vi "process_exit_callback.vi"(4 "ProcessExit Event":refnum<user-event>, 5 "Event Data":cluster{"sender":refnum<k24>, "e":refnum<k24>}, 6 "Control Ref":refnum<k24>, 7 "Event Common Data":T1) -> ()   [LabVIEW 2021, in "dotnet_system_exec.lvclass"]
doc: "Process Exit Callback VI"
uses:
  dotnet_system_exec.lvclass
  ProcessExit Event.ctl
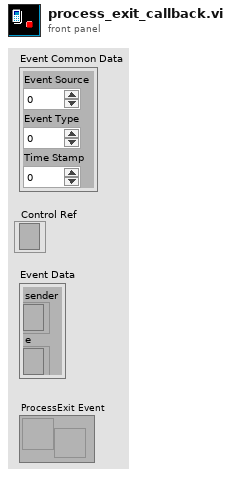
[diagram p1: front panel]
types:
  T1 = cluster{"Event Source":i32, "Event Type":u32, "Time Stamp":u32}
  T2 = typedef "dotnet_system_exec.lvclass/ProcessExit Event.ctl" = cluster{"HasExited":bool, "ExitCode":i32}
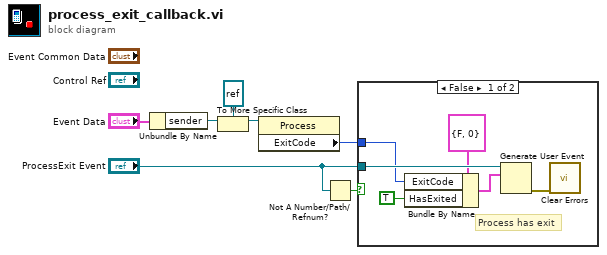
[diagram p0: block diagram]
diagram:
  n1 = Unbundle By Name("Event Data") -> ("sender"=w1:refnum<k24>)
  n2 = To More Specific Class(target class=refnum<k24> refnum ("Process Ref"), reference=w1) -> (specific class reference=w4:refnum<k24>)  [unwired: 1 in, 1 out]
  n3 = property class="Process"(reference=w4) -> ("ExitCode"=w2:i32)  [unwired: 1 in, 2 out]
  n4 = Not A Number/Path/Refnum?(number/path/refnum="ProcessExit Event") -> (NaN/Path/Refnum?=w7:bool)
  n5 = case shown="False" w7 {
    tunnel: "ProcessExit Event" -> [w13 _]
    tunnel: w2 -> [w9 _]
    frame False {
      # "Process has exit"
      n6 = Bundle By Name(cluster=T2 {"HasExited"=FALSE, "ExitCode"=0} ("ProcessExit Event"), "ExitCode"=w9, "HasExited"=TRUE ("event data")) -> (w10:T2)
      n7 = Generate User Event(user event=w13, event data cluster=w10) -> (error out=w12:errorcluster)  [unwired: 2 in, 1 out]
      n8 = call <vilib>:"Clear Errors.vi"("error in (no error)"=w12) -> ()  [unwired: 5 in, 2 out]
    }
    frame True {
    }
  }
